vi "Check_user.vi"(8 "error in (no error)":errorcluster, 9 "Enum":T1, 10 "Password":string, 11 "Name":string) -> (0 "error out":errorcluster, 3 "Result":bool)   [LabVIEW 2021]
uses:
  Control/login_type.ctl
  <vilib>/regexp/Match Regular Expression.xnode
panel:
  out "Application Directory":path
  out "concatenated string":string
  out "standard output":string
  out "standard error":string
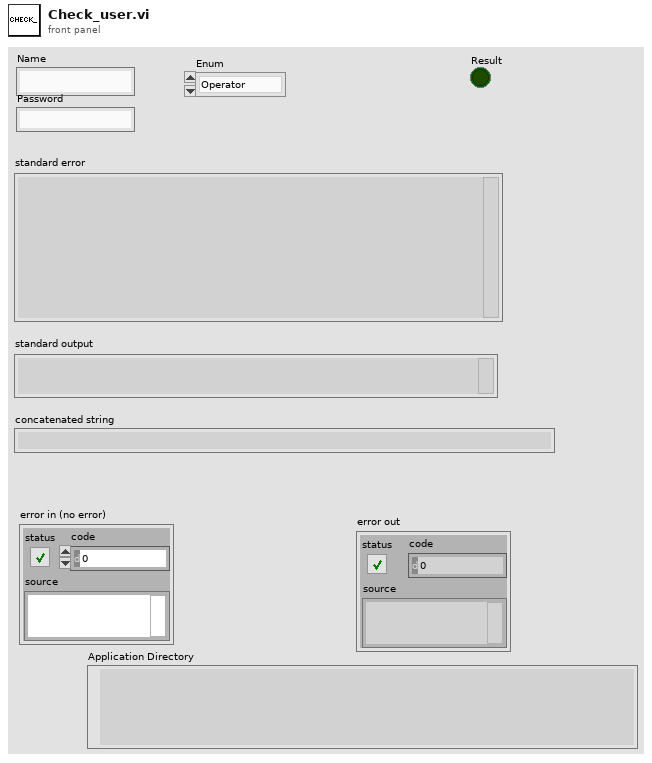
[diagram p1: front panel]
types:
  T1 = typedef "login_type.ctl" = enum16{"Operator", "Admin"}
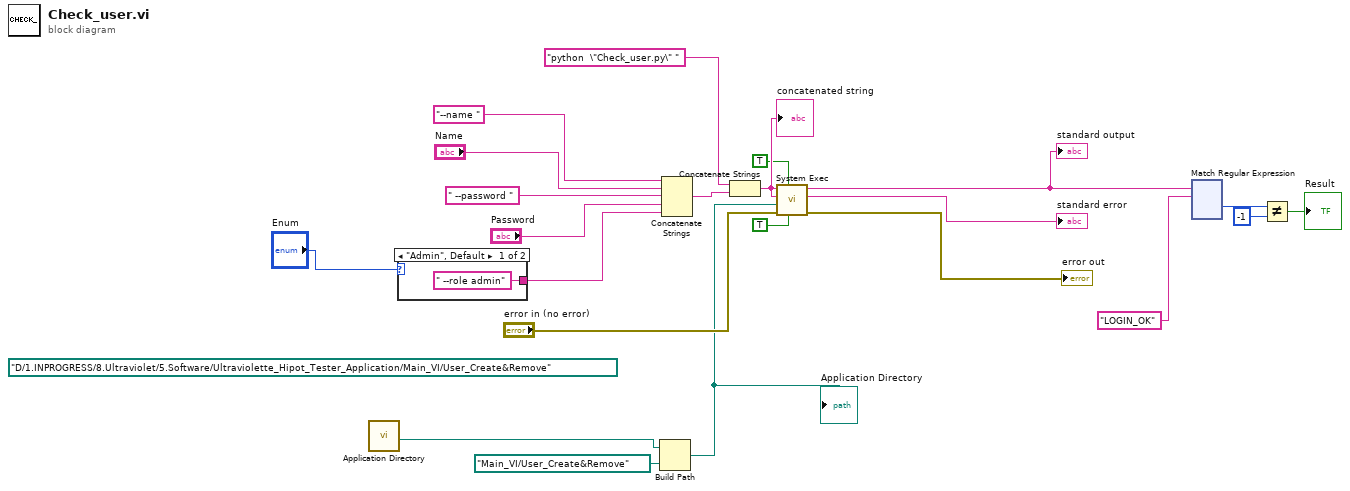
[diagram p0: block diagram]
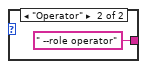
[diagram p2: hidden frame]
diagram:
  (unwired) path "D:/1.INPROGRESS/8.Ultraviolet/5.Software/Ultraviolette_Hipot_Tester_Application/Main_VI/User_Create&Remove" ("working directory")
  n1 = call <vilib>:"Application Directory.vi"() -> ("Application Directory"=w3:path)
  n2 = case shown="\"Admin\", Default" "Enum" {
    tunnel: [" --role admin" ("string") " --role operator" ("string")] -> w6
    frame "Admin", Default {
    }
    frame "Operator" {
    }
  }
  n3 = Build Path(base path=w3, name or relative path=path "Main_VI/User_Create&Remove") -> (appended path=w1:path)
  "Application Directory" <- w1
  n4 = Concatenate Strings("--name " ("string"), "Name", " --password " ("standard input"), "Password", w6) -> (w14:string)
  n5 = Concatenate Strings("python  \"Check_user.py\" " ("command line"), w14) -> (w20:string)
  "concatenated string" <- w20
  n6 = call <vilib>:"System Exec.vi"("run minimized? (F)"=TRUE, "wait until completion? (T)"=TRUE, "error in (no error)"="error in (no error)", "working directory"=w1, "standard input"=w20, "command line"=w20) -> ("error out"=→"error out":errorcluster, "standard error"=→"standard error":string, "standard output"=w13:string)  [unwired: 2 in, 1 out]
  "standard output" <- w13
  n7 = xnode "Match Regular Expression"("input string"=w13, "regular expression"="LOGIN_OK") -> ("offset past match"=w11:i32)  [unwired: 4 in, 4 out]
  n8 = Not Equal?(x=w11, y=-1) -> (x != y?=→"Result":bool)
